vi "Tell Self.vi"(4 "Priority":bool, 7 "Actor in":refnum<class "Actor.lvclass">, 8 "Error in":errorcluster, 9 "Reply":bool, 10 "Msg":refnum<class "Msg.lvclass">) -> (0 "Error out":errorcluster, 5 "Actor out":refnum<class "Actor.lvclass">)   [LabVIEW 2020, in "jettl.lvlib"]
uses:
  jettl.lvlib
  Msg/Msg.lvclass
  Actor/Actor.lvclass
  Relation.ctl
  Base Teller/Base Teller/Base Teller.lvclass/Base Teller.ctl
  Default Implementation.vi
  Base Teller/Init Teller.vi
  Base Teller/Base Teller/Init Teller.vi
  Base Teller/Base Teller/Base Teller.lvclass
  C:/git/jettl/src/jettl/jettl/Teller/Teller.lvclass
  Attributes/Attributes.lvclass
  Msg Input/Msg Input.lvclass
  Transport/Transport.lvclass
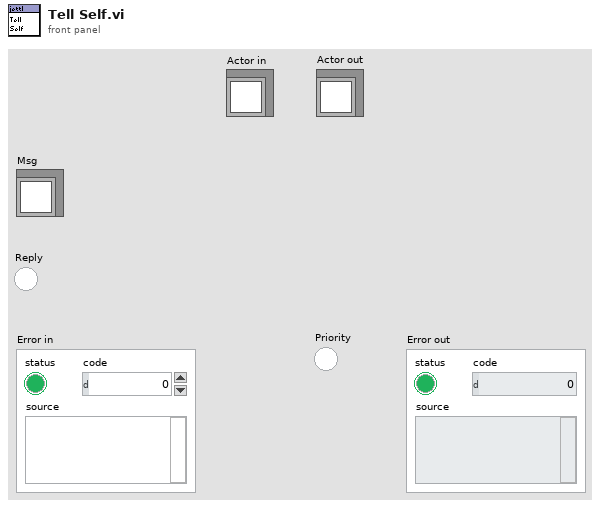
[diagram p1: front panel]
types:
  T1 = typedef "jettl.lvlib/Relation.ctl" = enum16{"Self", "Parent", "Child", "No Relation"}
  T2 = typedef "jettl.lvlib/Msgs.ctl" = set{refnum<class "Msg.lvclass">}
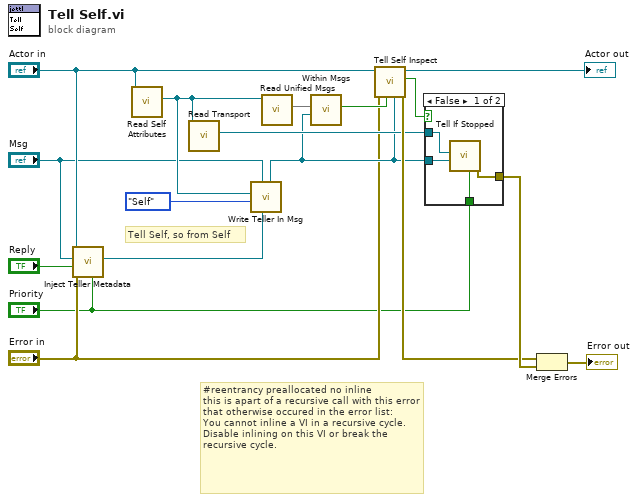
[diagram p0: block diagram]
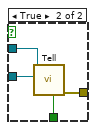
[diagram p2: hidden frame]
diagram:
  # "#reentrancy preallocated no inline\nthis is apart of a recursive call with this error that otherwise occured in the error list:\nYou cannot inline a VI in a recursive cycle. Disable inlining on this VI or break the recursive cycle."
  # "Tell Self, so from Self"
  n1 = call-dynamic "Inject Teller Metadata.vi"("Priority"="Priority", "Error in"="Error in", "Reply"="Reply", "Msg"="Msg", "Actor in"="Actor in") -> ("Teller Metadata"=w5:refnum<class "Teller Metadata.lvclass">)  [unwired: 6 in]
  n2 = call-dynamic "Read Self Attributes.vi"("Actor in"="Actor in") -> ("Self Attributes"=w7:refnum<class "Attributes.lvclass">)  [unwired: 10 in]
  n3 = call-dynamic "Read Transport.vi"("Attributes in"=w7) -> ("Transport"=w12:refnum<class "Transport.lvclass">)  [unwired: 10 in]
  n4 = call "Write Teller In Msg.vi"("Teller Metadata"=w5, "Msg in"="Msg", "Relation"=Relation."Self", "Attributes"=w7) -> ("Msg out"=w9:refnum<class "Msg.lvclass">)  [unwired: 7 in]
  n5 = call-dynamic "Read Unified Msgs.vi"("Attributes in"=w7) -> ("Unified Msgs"=w16:T2)  [unwired: 10 in]
  n6 = call "Within Msgs.vi"("Msg"=w9, "Msgs"=w16) -> ("Within Msgs"=w8:bool)  [unwired: 9 in]
  n7 = call-dynamic "Tell Self Inspect.vi"("Msg"=w9, "Within Unified Msgs"=w8, "Error in"="Error in", "Actor in"="Actor in") -> ("Error out"=w13:errorcluster, "Proceed"=w10:bool, "Actor out"=→"Actor out":refnum<class "Actor.lvclass">)  [unwired: 5 in]
  n8 = case shown="False" w10 {
    tunnel: [w18 w25] -> w17
    tunnel: w12 -> [w21 w24]
    tunnel: w9 -> [w20 w23]
    tunnel: "Priority" -> [w19 w22]
    frame False {
      n9 = call "Tell If Stopped.vi"("Priority"=w19, "Msg"=w20, "Transport"=w21) -> ("Error out"=w18:errorcluster)  [unwired: 8 in]
    }
    frame True {
      n10 = call-dynamic "Tell.vi"("Priority"=w22, "Msg"=w23, "Transport in"=w24) -> ("Error out"=w25:errorcluster)  [unwired: 8 in]
    }
  }
  n11 = Merge Errors(w13, w17) -> (→"Error out":errorcluster)
